vi "Tree.vi"() -> ()   [LabVIEW 2019]
uses:
  LV-Data/Typedefs/Dictionary--cluster.ctl
  LV-Data/Typedefs/File Type--enum.ctl
  LV-Data/LV-Data.lvclass
  LV-Data.ITX/LV-Data.ITX.lvclass
  LV-Data.ITX/ITX Commands/ITX Commands.lvclass
  LV-Data.DAT/LV-Data.DAT.lvclass
  LV-Data.TDMS/LV-Data.TDMS.lvclass
  Macros/Conversion.lvclass
  LV-Data/API/XY-Data to Dictionary (single).vi
  LV-Data/API/XY-Data to Dictionary (Multiple).vi
  LV-Data/Typedefs/Operation--enum.ctl
  LV-Data.DAT/Write DAT (1D).vi
panel:
  in  "Append Index":i32
  in  "File Type":T1
  in  "error in (no error)":errorcluster
  in  "Notes":string
  in  "Data (Dictionary)":T2[](array[typedef])
  in  "path":path
  out "path out":path
  out "Data (Dictionary) out":T2[](array[typedef])
  out "Notes out":string
  out "error out":errorcluster
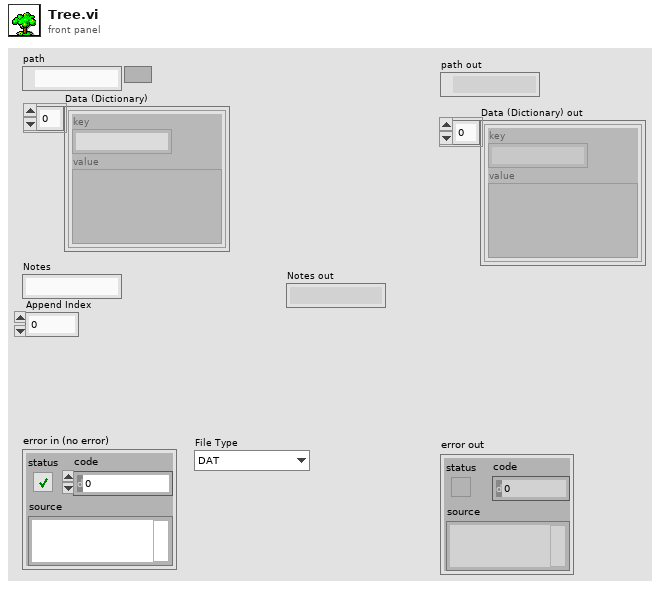
[diagram p1: front panel]
types:
  T1 = typedef "LV-Data.lvclass/File Type--enum.ctl" = enum16{"DAT", "ITX", "TDMS", "VI"}
  T2 = typedef "LV-Data.lvclass/Dictionary--cluster.ctl" = cluster{"key":string, "value":variant}
  T3 = typedef "LV-Data.lvclass/Operation--enum.ctl" = enum16{"Read", "Write", "Write + Append"}
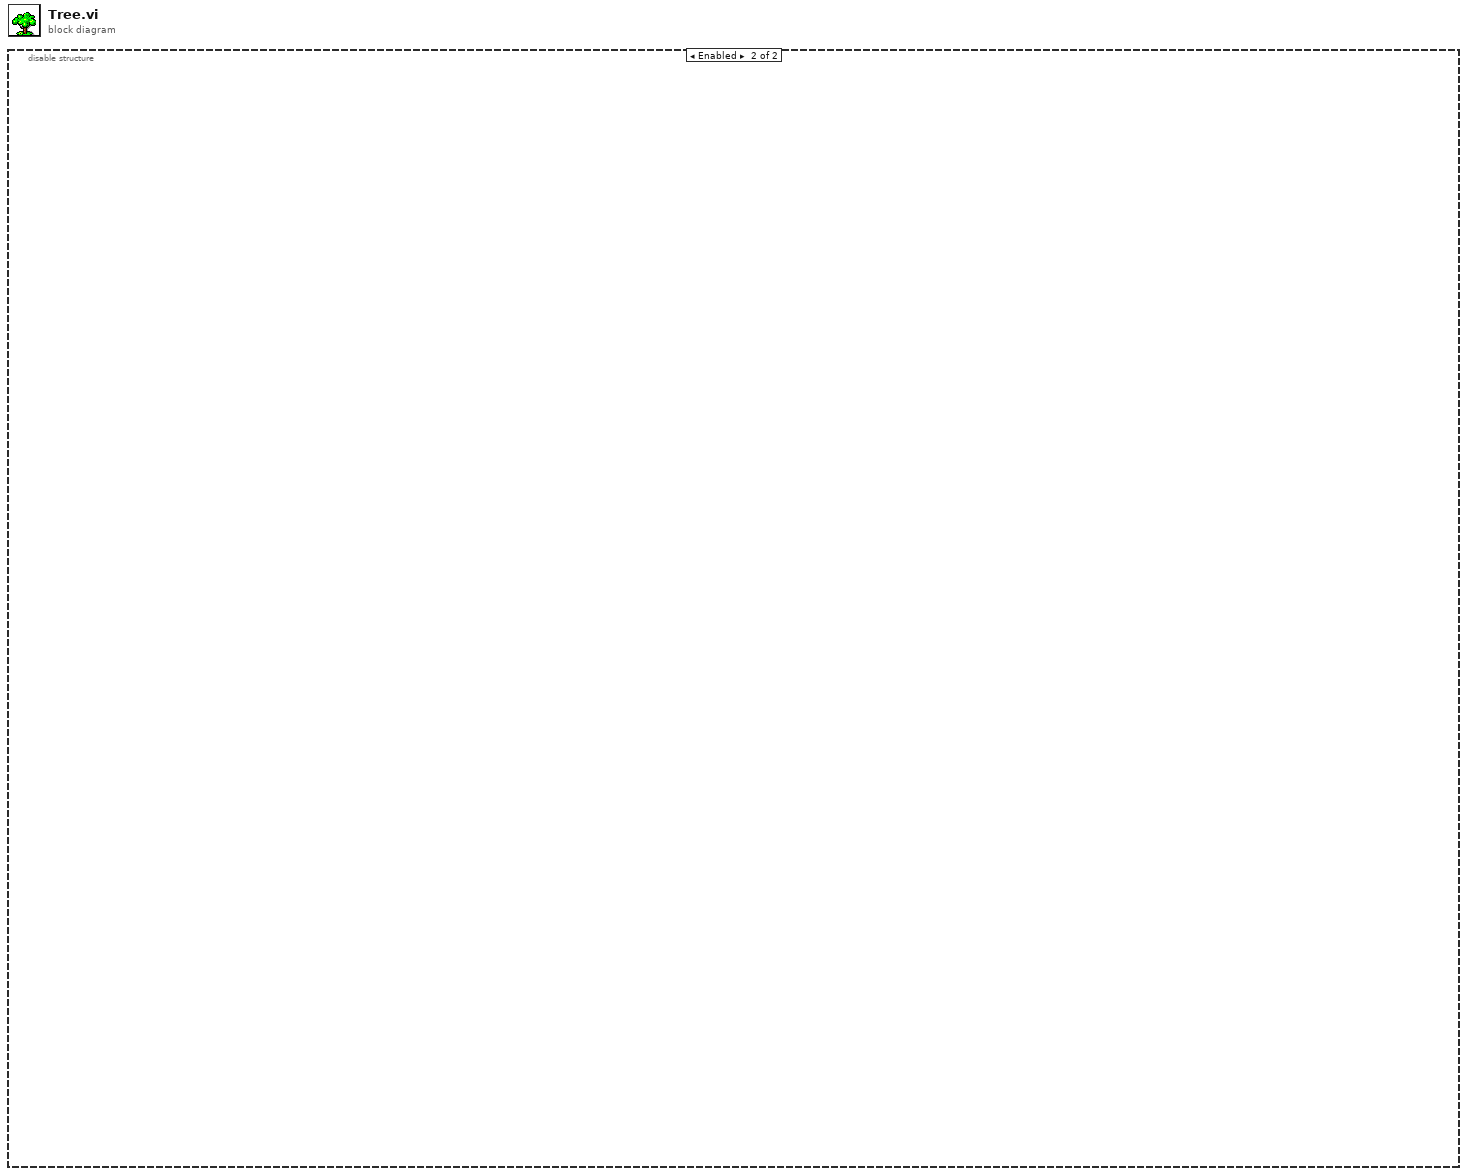
[diagram p0: block diagram]
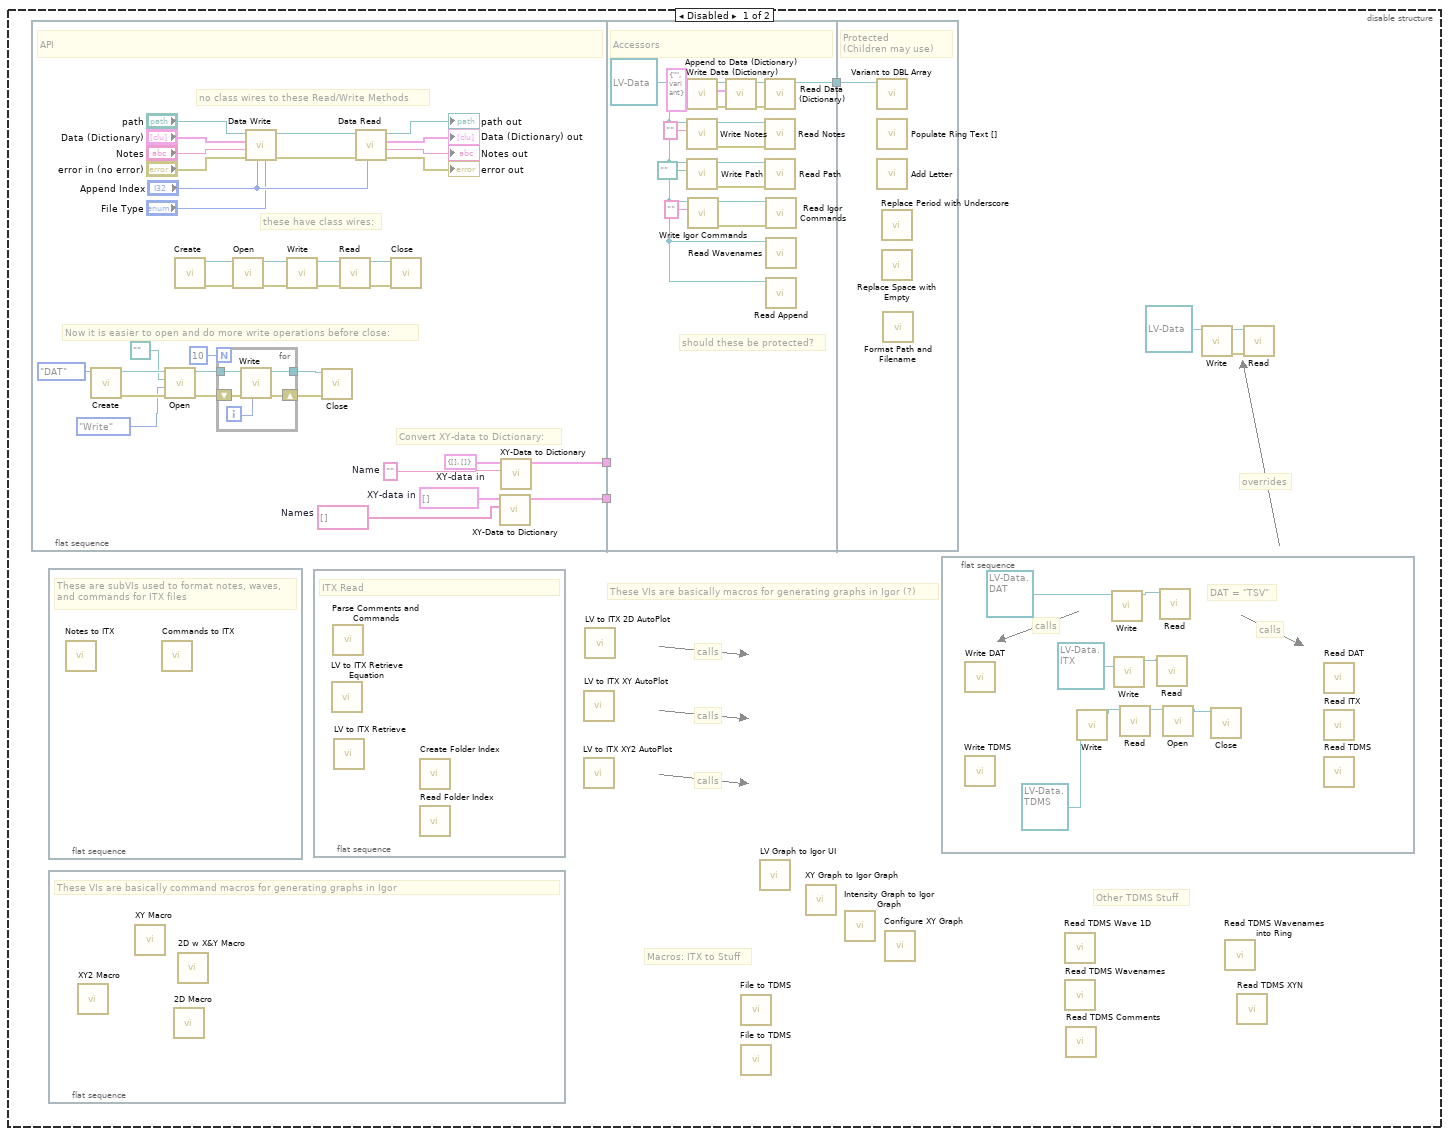
[diagram p2: hidden frame]
diagram:
  n1 = disable-structure shown="Enabled" {
    frame Disabled {
      # "calls"
      # "calls"
      # "calls"
      # "overrides"
      # "Macros: ITX to Stuff"
      # "Other TDMS Stuff"
      # "These VIs are basically macros for generating graphs in Igor (?)"
      n2 = flat-sequence {
        tunnel: [w42] -> w6
        tunnel: [w40] -> w5
        tunnel: w6 -> [_]
        tunnel: w5 -> [_]
        tunnel: [w60] -> w3
        tunnel: w3 -> [w72]
        frame #0 {
          w38 = string[] []  # Names
          w39 = ""  # Name
          w41 = cluster{"X-array":dbl[], "Y-array":dbl[]}[] []  # XY-data in
          w43 = cluster{"X-array":dbl[], "Y-array":dbl[]} {"X-array"=[], "Y-array"=[]}  # XY-data in
          # "Now it is easier to open and do more write operations before close:"
          # "Convert XY-data to Dictionary:"
          # "these have class wires:"
          # "no class wires to these Read/Write Methods"
          # "API"
          n3 = call "Create.vi"("File Type"=File_Type--enum."DAT") -> ("error out"=w29:errorcluster, "Data out"=w28:refnum<class "LV-Data.lvclass">)  [unwired: 9 in]
          n4 = call-dynamic "Open.vi"("error in (no error)"=w29, "Operation"=Operation--enum."Write", "Path"=path "", "Data in"=w28) -> ("error out"=w27:errorcluster, "Data out"=w26:refnum<class "LV-Data.lvclass">)  [unwired: 6 in]
          n5 = call "Create.vi"() -> ("error out"=w36:errorcluster, "Data out"=w37:refnum<class "LV-Data.lvclass">)  [unwired: 10 in]
          n6 = for {
            N: 10 -> [_]
            tunnel: w26 -> [w53]
            tunnel: [w51] -> w24
            shift-right: [w52] -> w25
            shift-left: w27 -> [w54]
            i -> [w55]
            n7 = call-dynamic "Write.vi"("Append Index"=w55, "error in (no error)"=w54, "Data in"=w53) -> ("error out"=w52:errorcluster, "Data out"=w51:refnum<class "LV-Data.lvclass">)  [unwired: 6 in, 1 out]
          }
          n8 = call-dynamic "Open.vi"("error in (no error)"=w36, "Data in"=w37) -> ("error out"=w34:errorcluster, "Data out"=w35:refnum<class "LV-Data.lvclass">)  [unwired: 8 in]
          n9 = call "Data Write.vi"("File Type"="File Type", "Append Index"="Append Index", "error in (no error)"="error in (no error)", "Notes"="Notes", "Data (Dictionary)"="Data (Dictionary)", "path"="path") -> ("error out"=w49:errorcluster, "path out"=w21:path)  [unwired: 4 in]
          n10 = call-dynamic "Write.vi"("error in (no error)"=w34, "Data in"=w35) -> ("error out"=w32:errorcluster, "Data out"=w33:refnum<class "LV-Data.lvclass">)  [unwired: 7 in, 1 out]
          n11 = call-dynamic "Close.vi"("error in (no error)"=w25, "Data in"=w24) -> ()  [unwired: 8 in, 2 out]
          n12 = call-dynamic "Read.vi"("error in (no error)"=w32, "Data Save in"=w33) -> ("error out"=w30:errorcluster, "Data Save out"=w31:refnum<class "LV-Data.lvclass">)  [unwired: 5 in, 3 out]
          n13 = call "Data Read.vi"("Append Index"="Append Index", "error in (no error)"=w49, "path"=w21) -> ("error out"=→"error out":errorcluster, "Notes"=→"Notes out":string, "Data (Dictionary)"=→"Data (Dictionary) out":T2[], "path out"=→"path out":path)  [unwired: 5 in]
          n14 = call-dynamic "Close.vi"("error in (no error)"=w30, "Data in"=w31) -> ()  [unwired: 8 in, 2 out]
          n15 = call-poly "XY-Data to Dictionary.vi"("Names"=w38, "XY-data in"=w41) -> ("Data (Dictionary)"=w40:T2[])  [unwired: 8 in, 1 out]
          n16 = call-poly "XY-Data to Dictionary.vi"("Name"=w39, "XY-data in"=w43) -> ("Data (Dictionary)"=w42:T2[])  [unwired: 8 in, 1 out]
        }
        frame #1 {
          w71 = refnum<class "LV-Data.lvclass"> refnum ("Data Save")
          # "should these be protected?"
          # "Accessors"
          n17 = call "Write Data (Dictionary).vi"("Data Save"=w71) -> ("error out"=w69:errorcluster, "Data Save out"=w70:refnum<class "LV-Data.lvclass">)  [unwired: 9 in]
          n18 = call "Write Notes.vi"("Notes"="", "Data Save"=w71) -> ("error out"=w65:errorcluster, "Data Save out"=w66:refnum<class "LV-Data.lvclass">)  [unwired: 8 in]
          n19 = call "Write Path.vi"("Path"=path "", "Data Save"=w71) -> ("error out"=w63:errorcluster, "Data Save out"=w64:refnum<class "LV-Data.lvclass">)  [unwired: 8 in]
          n20 = call "Write Igor Commands.vi"("Igor Commands"="", "Data Save"=w71) -> ("error out"=w61:errorcluster, "Data Save out"=w62:refnum<class "LV-Data.lvclass">)  [unwired: 8 in]
          n21 = call "Append to Data (Dictionary).vi"("error in (no error)"=w69, "key-value"=cluster{"key":string, "value":variant} {"key"="", "value"=variant}, "Data Save"=w70) -> ("error out"=w67:errorcluster, "Data Save out"=w68:refnum<class "LV-Data.lvclass">)  [unwired: 7 in]
          n22 = call "Read Data (Dictionary).vi"("error in (no error)"=w67, "Data Save"=w68) -> ("Data Save out"=w60:refnum<class "LV-Data.lvclass">)  [unwired: 7 in, 2 out]
          n23 = call "Read Notes.vi"("error in (no error)"=w65, "Data Save"=w66) -> ()  [unwired: 7 in, 3 out]
          n24 = call "Read Path.vi"("error in (no error)"=w63, "Data Save"=w64) -> ()  [unwired: 7 in, 3 out]
          n25 = call "Read Igor Commands.vi"("error in (no error)"=w61, "Data Save"=w62) -> ()  [unwired: 7 in, 3 out]
          n26 = call "Read Wavenames.vi"("Data Save"=w71) -> ()  [unwired: 8 in, 3 out]
          n27 = call "Read Append.vi"("Data in"=w71) -> ()  [unwired: 8 in, 3 out]
        }
        frame #2 {
          # "Protected\n(Children may use)"
          n28 = call "Variant to DBL Array.vi"("Data (Variant)"=w72) -> ()  [unwired: 8 in, 3 out]
          n29 = call "Populate Ring Text [].vi"() -> ()  [unwired: 11 in, 1 out]
          n30 = call "Add Letter.vi"() -> ()  [unwired: 1 in, 1 out]
          n31 = call "Replace Period with Underscore.vi"() -> ()  [unwired: 1 in, 1 out]
          n32 = call "Replace Space with Empty.vi"() -> ()  [unwired: 1 in, 1 out]
          n33 = call "Format Path and Filename.vi"() -> ()  [unwired: 10 in, 2 out]
        }
      }
      n34 = flat-sequence {
        frame #0 {
          # "These are subVIs used to format notes, waves, and commands for ITX files"
          n35 = call "Notes to ITX.vi"() -> ()  [unwired: 1 in, 1 out]
          n36 = call "Commands to ITX.vi"() -> ()  [unwired: 1 in, 1 out]
        }
      }
      n37 = flat-sequence {
        frame #0 {
          # "These VIs are basically command macros for generating graphs in Igor"
          n38 = call "XY2 Macro.vi"() -> ()  [unwired: 9 in, 3 out]
          n39 = call "XY Macro.vi"() -> ()  [unwired: 9 in, 3 out]
          n40 = call "2D Macro.vi"() -> ()  [unwired: 9 in, 3 out]
          n41 = call "2D w X&Y Macro.vi"() -> ()  [unwired: 13 in, 3 out]
        }
      }
      n42 = flat-sequence {
        frame #0 {
          # "ITX Read"
          n43 = call "LV to ITX Retrieve Equation.vi"() -> ()  [unwired: 11 in, 5 out]
          n44 = call "Parse Comments and Commands.vi"() -> ()  [unwired: 2 in, 2 out]
          n45 = call "LV to ITX Retrieve.vi"() -> ()  [unwired: 11 in, 5 out]
          n46 = call "Create Folder Index.vi"() -> ()  [unwired: 11 in, 1 out]
          n47 = call "Read Folder Index.vi"() -> ()  [unwired: 10 in, 2 out]
        }
      }
      n48 = call "LV to ITX XY AutoPlot.vi"() -> ()  [unwired: 10 in, 2 out]
      n49 = call "LV to ITX XY2 AutoPlot.vi"() -> ()  [unwired: 10 in, 2 out]
      n50 = call "LV to ITX 2D AutoPlot.vi"() -> ()  [unwired: 10 in, 2 out]
      n51 = call "File to TDMS.vi"() -> ()  [unwired: 9 in, 3 out]
      n52 = call "File to TDMS.vi"() -> ()  [unwired: 9 in, 3 out]
      n53 = call "LV Graph to Igor UI.vi"() -> ()  [unwired: 12 in]
      n54 = call "XY Graph to Igor Graph.vi"() -> ()  [unwired: 10 in, 2 out]
      n55 = call "Intensity Graph to Igor Graph.vi"() -> ()  [unwired: 10 in, 2 out]
      n56 = call "Configure XY Graph.vi"() -> ()  [unwired: 11 in, 1 out]
      n57 = flat-sequence {
        frame #0 {
          # "DAT = \"TSV\""
          # "calls"
          # "calls"
          n58 = call-poly "Write DAT.vi"() -> ()  [unwired: 10 in, 2 out]
          n59 = call "Write TDMS.vi"() -> ()  [unwired: 10 in, 2 out]
          n60 = call-dynamic "Write.vi"("Data.TDMS in"=refnum<class "LV-Data.TDMS.lvclass"> refnum) -> ("Data.TDMS out"=w9:refnum<class "LV-Data.TDMS.lvclass">)  [unwired: 8 in, 2 out]
          n61 = call-dynamic "Write.vi"("Data.DAT in"=refnum<class "LV-Data.DAT.lvclass"> refnum) -> ("Data.DAT out"=w13:refnum<class "LV-Data.DAT.lvclass">)  [unwired: 8 in, 2 out]
          n62 = call-dynamic "Write.vi"("Data.ITX in"=refnum<class "LV-Data.ITX.lvclass"> refnum) -> ("Data.ITX out"=w11:refnum<class "LV-Data.ITX.lvclass">)  [unwired: 8 in, 2 out]
          n63 = call-dynamic "Read.vi"("Data.TDMS"=w9) -> ("Data.TDMS out"=w8:refnum<class "LV-Data.TDMS.lvclass">)  [unwired: 6 in, 4 out]
          n64 = call-dynamic "Read.vi"("ITX"=w11) -> ()  [unwired: 6 in, 5 out]
          n65 = call-dynamic "Read.vi"("DAT in"=w13) -> ()  [unwired: 6 in, 5 out]
          n66 = call-dynamic "Open.vi"("Data.TDMS in"=w8) -> ("Data.TDMS out"=w7:refnum<class "LV-Data.TDMS.lvclass">)  [unwired: 9 in, 1 out]
          n67 = call-dynamic "Close.vi"("Data.TDMS in"=w7) -> ()  [unwired: 9 in, 2 out]
          n68 = call "Read DAT.vi"() -> ()  [unwired: 9 in, 3 out]
          n69 = call "Read ITX.vi"() -> ()  [unwired: 8 in, 4 out]
          n70 = call "Read TDMS.vi"() -> ()  [unwired: 8 in, 4 out]
        }
      }
      n71 = call "Read TDMS Wave 1D.vi"() -> ()  [unwired: 9 in, 3 out]
      n72 = call "Read TDMS Wavenames.vi"() -> ()  [unwired: 9 in, 3 out]
      n73 = call "Read TDMS Comments.vi"() -> ()  [unwired: 9 in, 3 out]
      n74 = call-dynamic "Write.vi"("Data in"=refnum<class "LV-Data.lvclass"> refnum) -> ("error out"=w4:errorcluster, "Data out"=w2:refnum<class "LV-Data.lvclass">)  [unwired: 8 in, 1 out]
      n75 = call "Read TDMS Wavenames into Ring.vi"() -> ()  [unwired: 11 in, 1 out]
      n76 = call "Read TDMS XYN.vi"() -> ()  [unwired: 9 in, 3 out]
      n77 = call-dynamic "Read.vi"("error in (no error)"=w4, "Data Save in"=w2) -> ()  [unwired: 5 in, 5 out]
    }
    frame Enabled {
    }
  }
